vi "Untitled 5.vi"   [LabVIEW 2026]
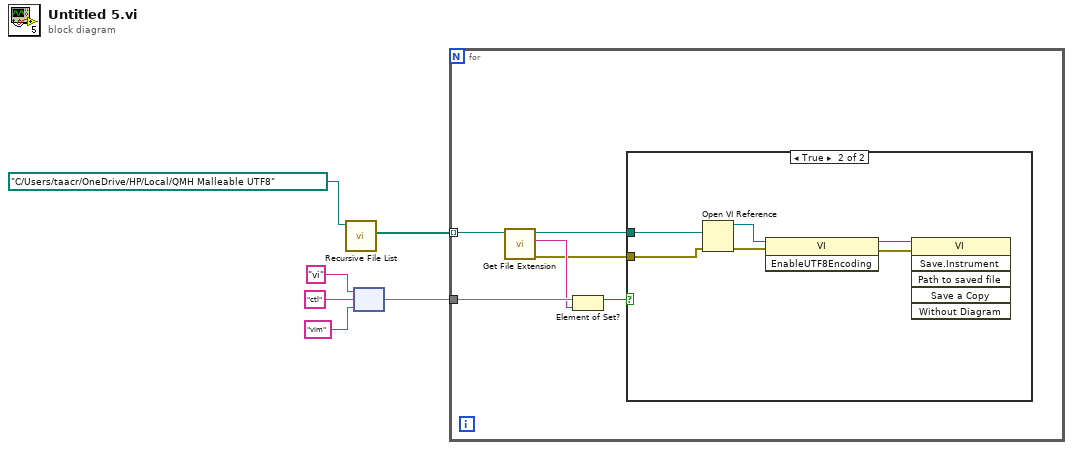
[diagram p0: block diagram]
diagram:
  n1 = call <vilib>:"Recursive File List.vi"("Folder Path"=path "C:/Users/taacr/OneDrive/HP/Local/QMH Malleable UTF8") -> ("All Files in Dir"=w5:path[])  [unwired: 6 in, 4 out]
  n2 = node("vi" ("String"), "ctl" ("String"), "vim" ("String")) -> (w1:set{string})
  n3 = for {
    tunnel: w5 -> [w12] mode=indexing
    tunnel: w1 -> [w11]
    n4 = call <vilib>:"Get File Extension.vi"("file"=w12) -> ("error out"=w7:errorcluster, "lowercase file extension"=w10:string, "dup file"=w9:path)  [unwired: 6 in, 2 out]
    n5 = Element of Set?(10:w10, 11:w11) -> (3:w8:bool)
    n6 = case shown="True" w8 {
      tunnel: w9 -> [_ w18]
      tunnel: w7 -> [_ w15]
      frame False {
      }
      frame True {
        n7 = Open VI Reference(vi path=w18, error in (no error)=w15) -> (vi reference=w17:refnum<vi>, error out=w16:errorcluster)  [unwired: 4 in]
        n8 = invoke class="VI" method="EnableUTF8Encoding"(reference=w17, error in=w16) -> (reference out=w14:refnum<vi>, error out=w13:errorcluster)  [unwired: 1 in, 1 out]
        n9 = invoke class="VI" method="Save.Instrument"(reference=w14, error in=w13) -> ()  [unwired: 4 in, 6 out]
      }
    }
  }
